vi "Iteration.vi"(7 "Variables in":refnum<class "Variables.lvclass">, 8 "error in (no error)":errorcluster, 9 "Timing":T1, 11 "State in":refnum<class "State.lvclass">) -> (0 "error out":errorcluster, 3 "State out":refnum<class "State.lvclass">, 5 "Variables":refnum<class "Variables.lvclass">)   [LabVIEW 2020, in "VolatusSeq.lvlib" / "State.lvclass"]
uses:
  State.lvclass
  Variables/Variables.lvclass
  Iteration Actions/Iteration Actions.lvclass
  Timing.ctl
  State.lvclass/State.ctl
  VolatusSeq.lvlib
panel:
  out "Actions":refnum<class "Iteration Actions.lvclass">
  in  "Actions In":refnum<class "Iteration Actions.lvclass">
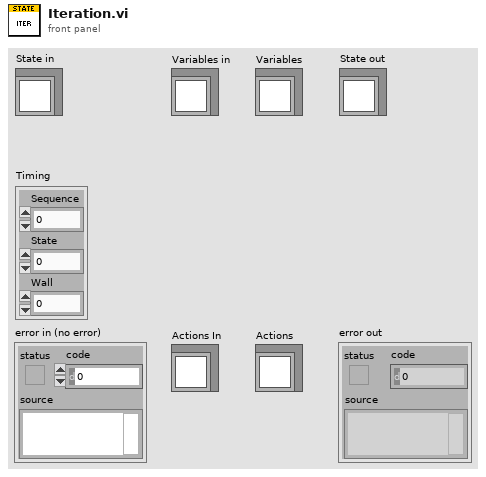
[diagram p1: front panel]
types:
  T1 = typedef "VolatusSeq.lvlib/Timing.ctl" = cluster{"Sequence":dbl, "State":dbl, "Wall":dbl}
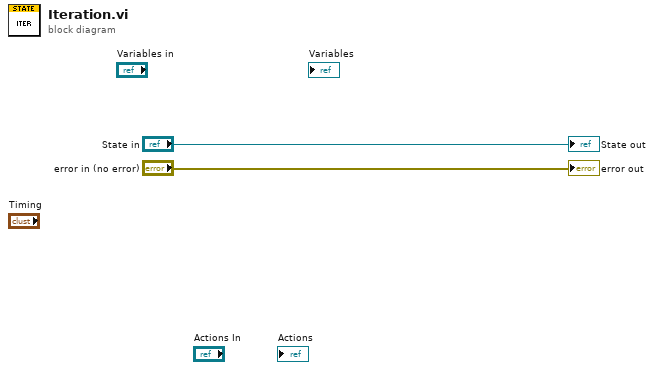
[diagram p0: block diagram]
diagram:
  "error out" <- "error in (no error)"
  "State out" <- "State in"
